vi "background writer.vi"(0 "dictionary":T1, 1 "command queue":refnum<k33>, 2 "response from processor":refnum<k33>, 3 "output type order":T3[](array[typedef]), 4 "File Property Indeces":i32[](array[numeric]), 5 "logging path":path, 7 "backup directory":path, 9 "cache allocation":T2, 10 "LogRotate":refnum<class "LogRotate.lvclass">=refnum, 11 "scans per write":u16=20, 12 "dictionary group names":T1, 13 "enable channel (bool)":i32, 14 "has enable channel":bool) -> (15 "error out":errorcluster)   [LabVIEW 2015, in "TDMS datalogger runtime.lvclass"]
uses:
  TDMS datalogger runtime.lvclass
  <vilib>/NI/Tag Bus/tag/Data Type.ctl
  data cache.ctl
  <vilib>/NI/Tag Bus/dictionary/full data dictionary.ctl
  message to background process.ctl
  control enum.ctl
  <vilib>/NI/Tag Bus/table/data table.ctl
  response from background process.ctl
  response enum.ctl
  <vilib>/NI/LogRotate/LogRotate.lvclass
  writer state enum.ctl
  <vilib>/NI/Tag Bus/table/data table.lvlib
  <vilib>/NI/Tag Bus/tag/tag descriptor.lvclass
  <vilib>/NI/Tag Bus/dictionary/data dictionary.lvclass
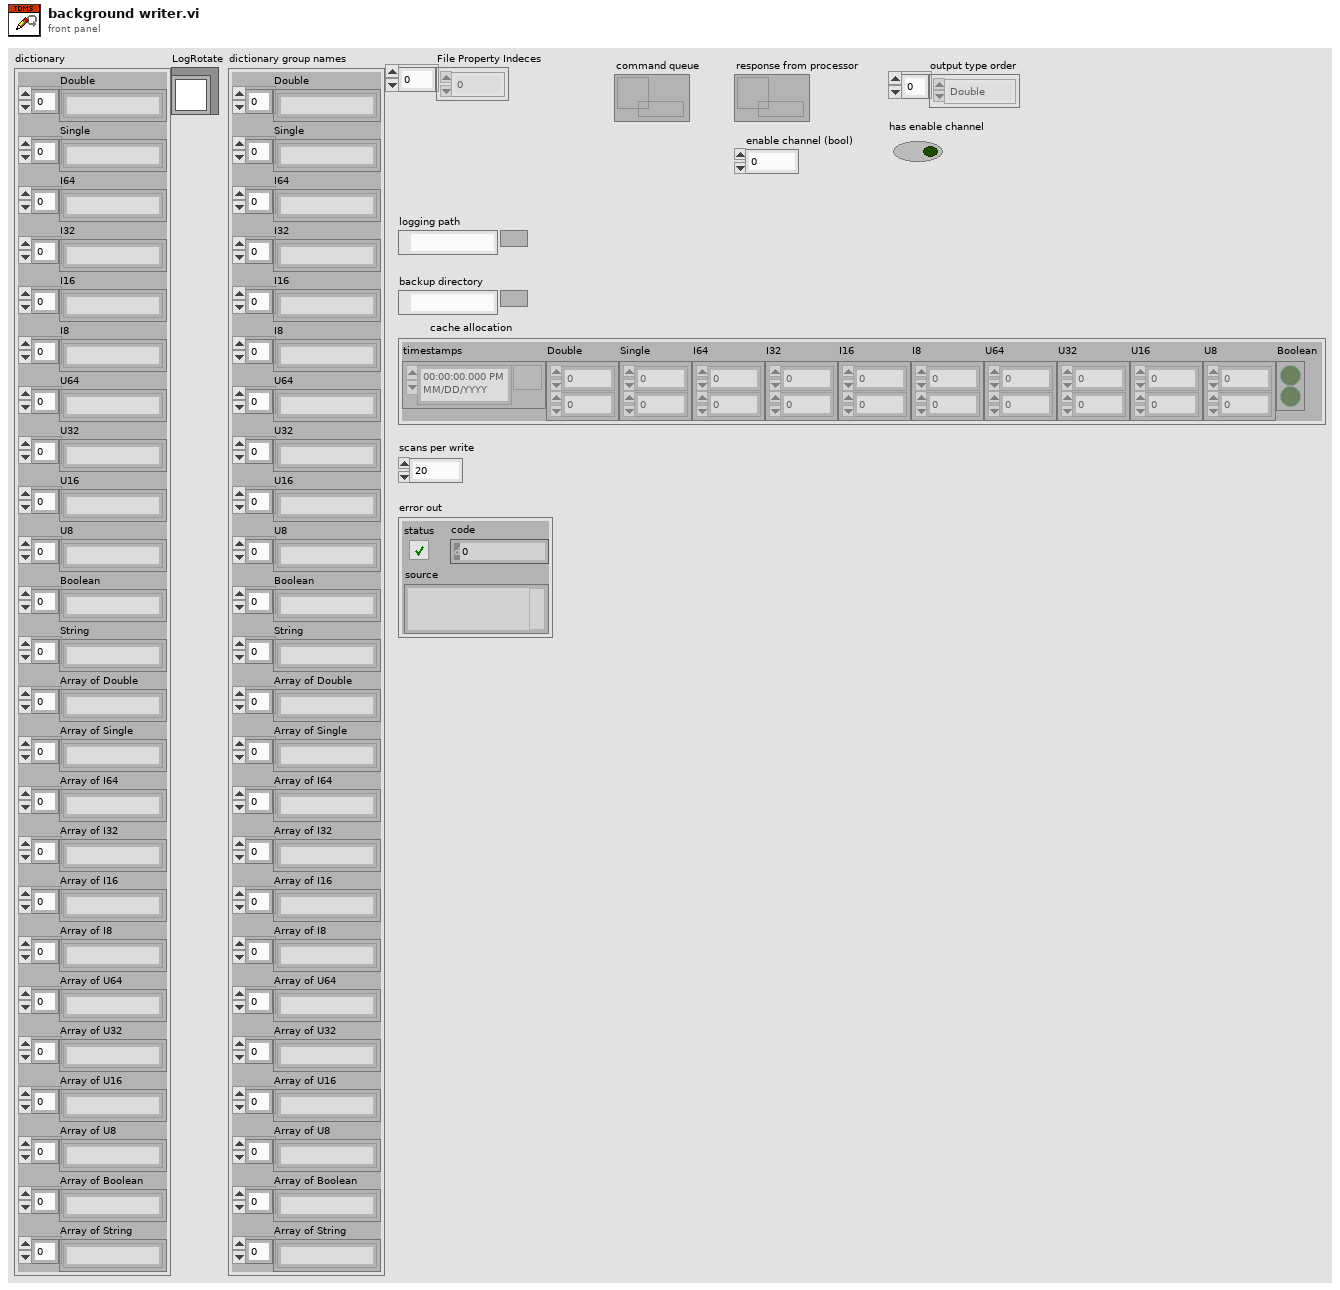
[diagram p1: front panel]
types:
  T1 = typedef "tag bus.lvlib/data dictionary.lvclass/full data dictionary.ctl" = cluster{"Double":string[], "Single":string[], "I64":string[], "I32":string[], "I16":string[], "I8":string[], "U64":string[], "U32":string[], "U16":string[], "U8":string[], "Boolean":string[], "String":string[], "Array of Double":string[], "Array of Single":string[], "Array of I64":string[], "Array of I32":string[], "Array of I16":string[], "Array of I8":string[], "Array of U64":string[], "Array of U32":string[], "Array of U16":string[], "Array of U8":string[], "Array of Boolean":string[], "Array of String":string[]}
  T2 = typedef "TDMS datalogger runtime.lvclass/data cache.ctl" = cluster{"timestamps":timestamp[], "Double":dbl[][], "Single":sgl[][], "I64":i64[][], "I32":i32[][], "I16":i16[][], "I8":i8[][], "U64":u64[][], "U32":u32[][], "U16":u16[][], "U8":u8[][], "Boolean":bool[][]}
  T3 = typedef "tag bus.lvlib/tag descriptor.lvclass/Data Type.ctl" = enum16{"Double", "Single", "I64", "I32", "I16", "I8", "U64", "U32", "U16", "U8", "Boolean", "String", "Array of Double", "Array of Single", "Array of I64", "Array of I32", "Array of I16", "Array of I8", "Array of U64", "Array of U32", "Array of U16", "Array of U8", "Array of Boolean", "Array of String"}
  T4 = typedef "TDMS datalogger runtime.lvclass/writer state enum.ctl" = enum16{"wait for message", "report error", "exit", "close file"}
  T5 = typedef "TDMS datalogger runtime.lvclass/response enum.ctl" = enum16{"exit", "return buffer", "error"}
  T6 = typedef "TDMS datalogger runtime.lvclass/response from background process.ctl" = cluster{"response enum":T5, "datapack":refnum<data-value>, "error code":i32}
  T7 = typedef "TDMS datalogger runtime.lvclass/message to background process.ctl" = cluster{"control enum":T8, "datapack":refnum<data-value>, "Time Stamp":timestamp}
  T8 = typedef "TDMS datalogger runtime.lvclass/control enum.ctl" = enum16{"exit", "output data"}
  T9 = typedef "tag bus.lvlib/data table.lvlib/data table.ctl" = cluster{"Double":dbl[], "Single":sgl[], "I64":i64[], "I32":i32[], "I16":i16[], "I8":i8[], "U64":u64[], "U32":u32[], "U16":u16[], "U8":u8[], "Boolean":bool[], "String":string[], "Array of Double":cluster{"DBL Array":dbl[]}[], "Array of Single":cluster{"SGL Array":sgl[]}[], "Array of I64":cluster{"I64 Array":i64[]}[], "Array of I32":cluster{"I32 Array":i32[]}[], "Array of I16":cluster{"I16 Array":i16[]}[], "Array of I8":cluster{"I8 Array":i8[]}[], "Array of U64":cluster{"U64 Array":u64[]}[], "Array of U32":cluster{"U32 Array":u32[]}[], "Array of U16":cluster{"U16 Array":u16[]}[], "Array of U8":cluster{"U8 Array":u8[]}[], "Array of Boolean":cluster{"Boolean Array":bool[]}[], "Array of String":cluster{"String Array":string[]}[]}
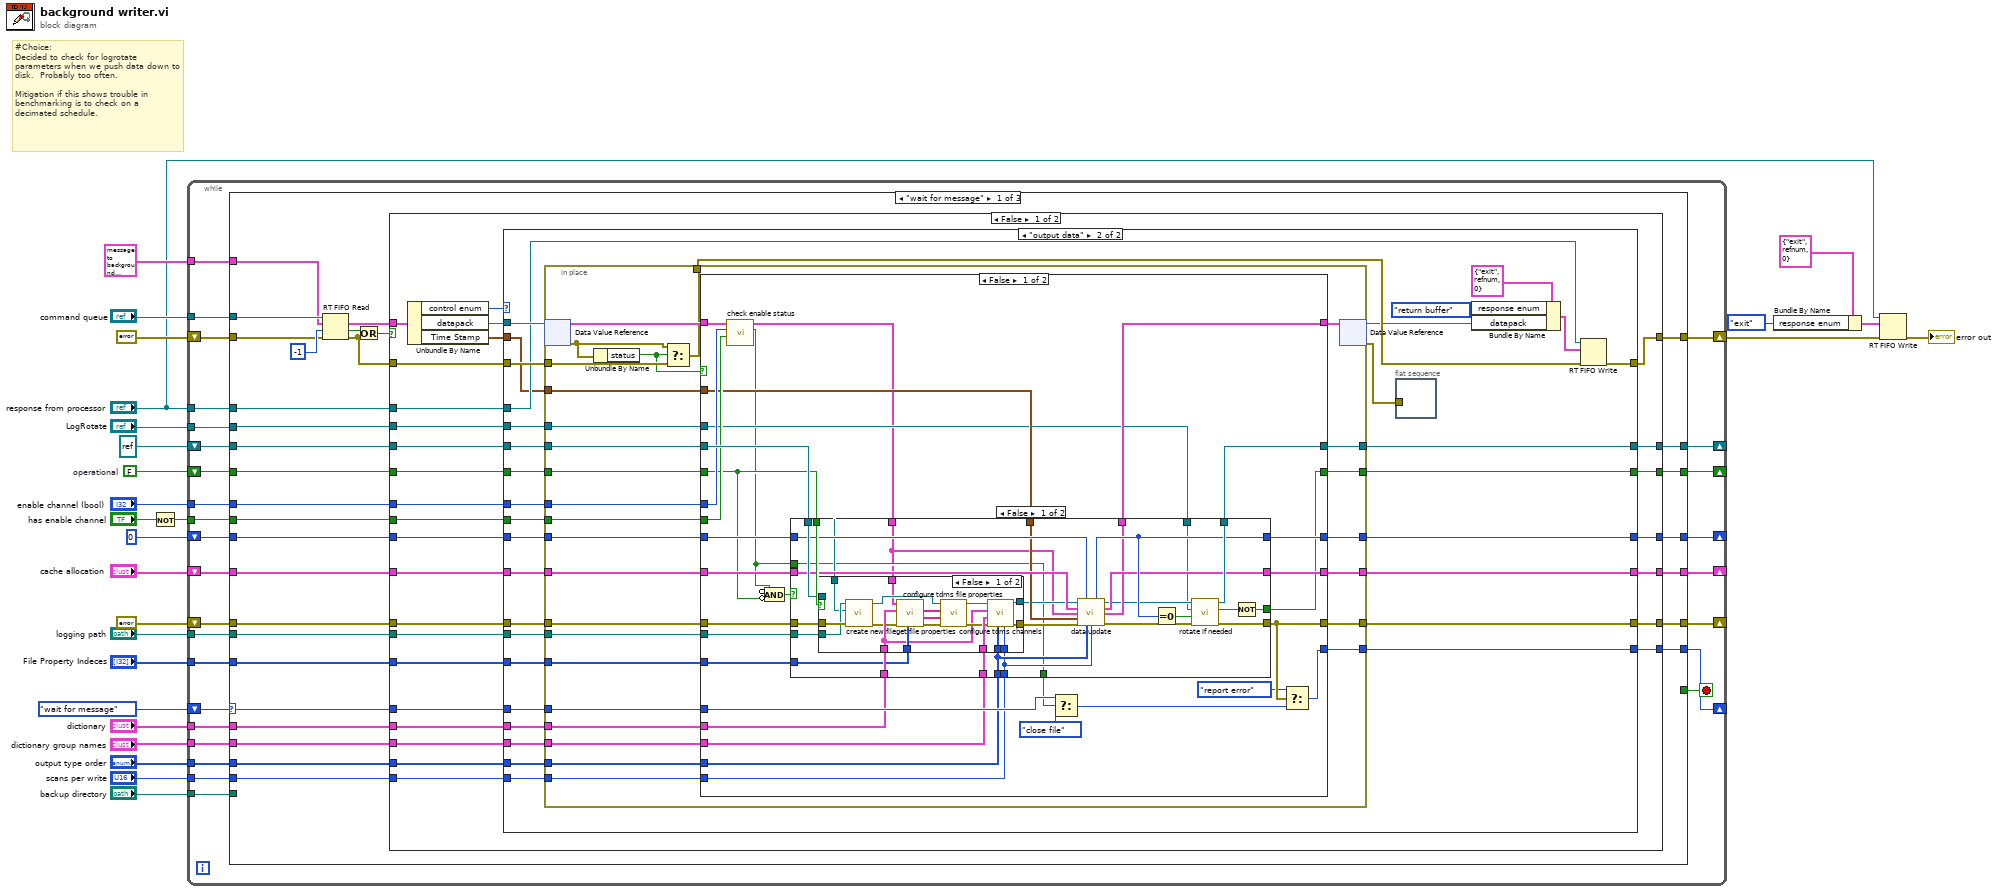
[diagram p0: block diagram]
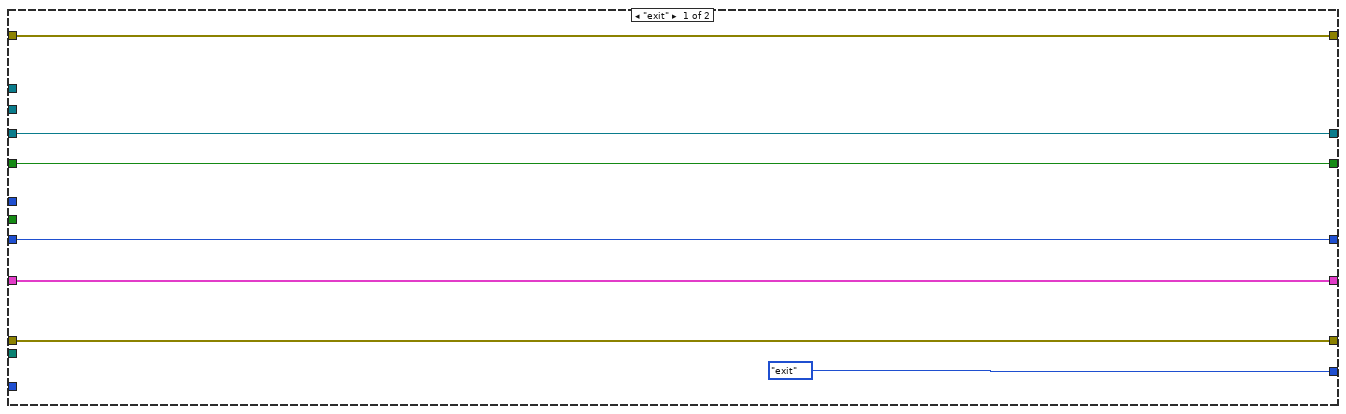
[diagram p2: hidden frame]
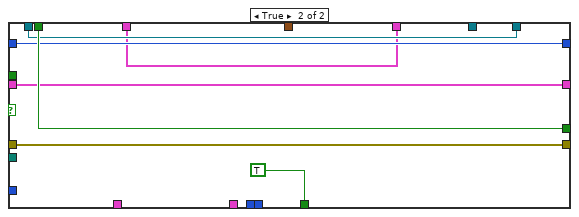
[diagram p4: hidden frame]
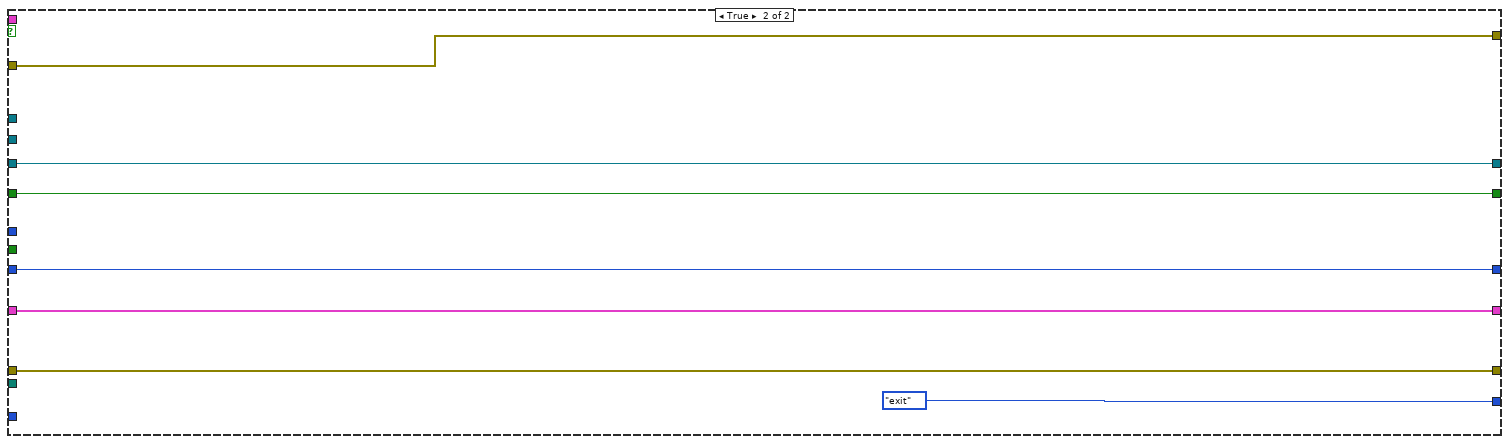
[diagram p6: hidden frame]
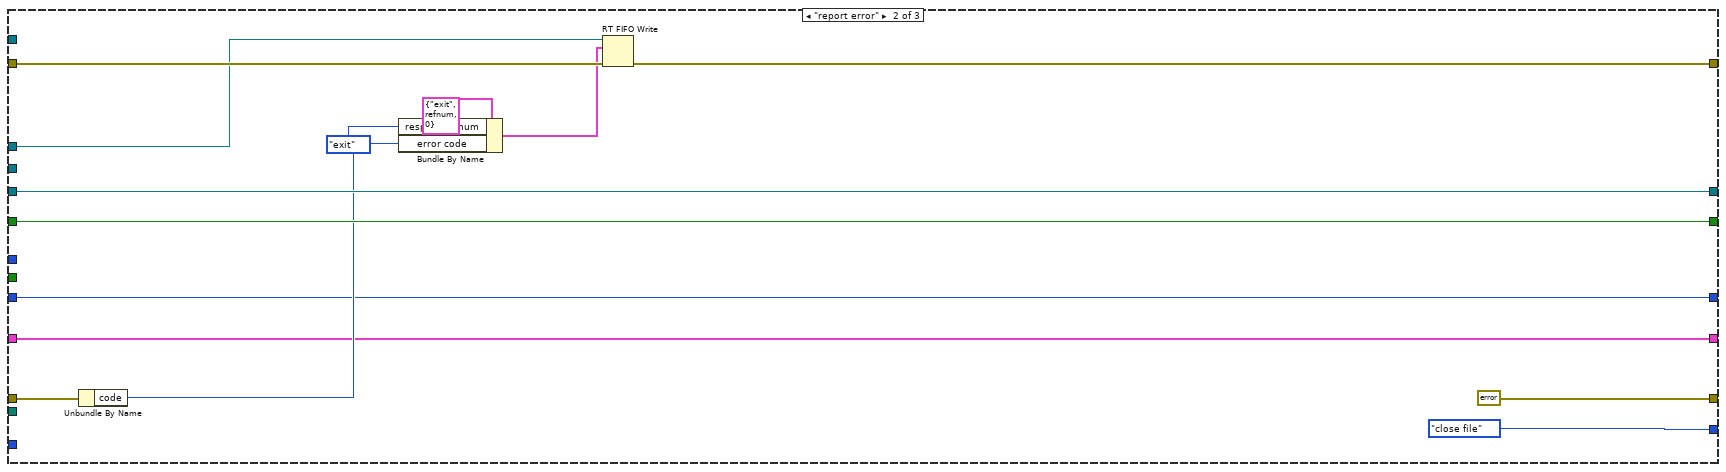
[diagram p7: hidden frame]
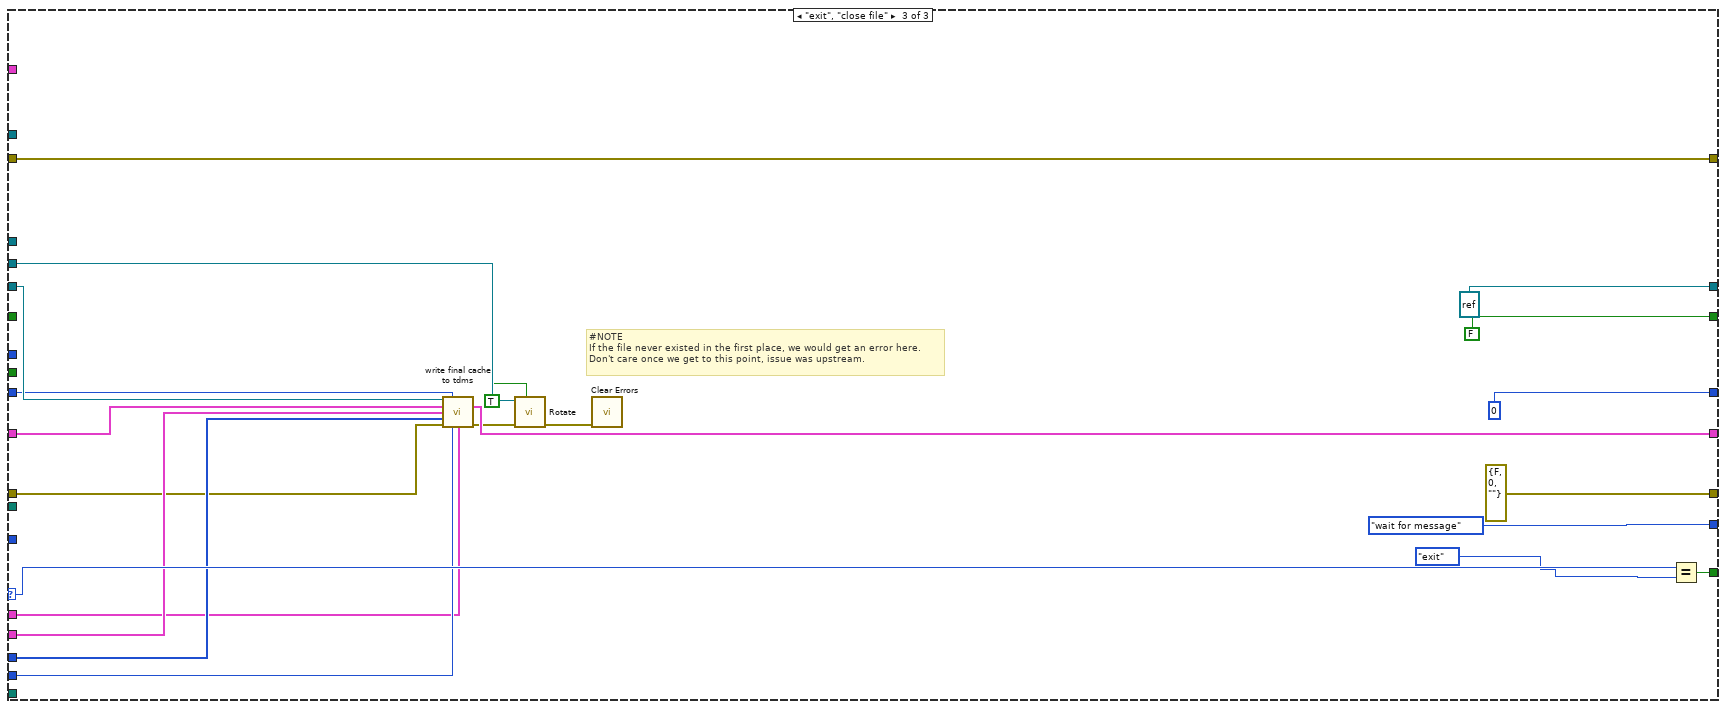
[diagram p8: hidden frame]
diagram:
  w15 = FALSE  # operational
  # "#Choice:\nDecided to check for logrotate parameters when we push data down to disk.  Probably too often.\n\nMitigation if this shows trouble in benchmarking is to check on a decimated schedule."
  n1 = Not(x="has enable channel") -> (.not. x?=w7:bool)
  n2 = while {
    tunnel: "command queue" -> [w54]
    tunnel: T7 {"control enum"=enum."exit", "datapack"=refnum, "Time Stamp"=timestamp(0 s since 1904-01-01)} ("element") -> [w53]
    shift-right: [w51] -> w23
    shift-left: errorcluster {"status"=FALSE, "code"=0, "source"=""} ("error in") -> [w52]
    tunnel: "response from processor" -> [w49]
    shift-right: [w47] -> _
    shift-left: writer_state_enum."wait for message" ("logger state") -> [w48]
    shift-right: [w45] -> _
    shift-left: refnum<k34> refnum ("tdms file out") -> [w46]
    shift-right: [w36] -> _
    shift-left: w15 -> [w44]
    shift-right: [w42] -> _
    shift-left: errorcluster {"status"=FALSE, "code"=0, "source"=""} ("error in") -> [w43]
    tunnel: "logging path" -> [w41]
    tunnel: "dictionary" -> [w40]
    tunnel: "output type order" -> [w39]
    tunnel: "scans per write" -> [w38]
    tunnel: "backup directory" -> [w37]
    shift-right: [w35] -> _
    shift-left: 0 ("sample counter") -> [w34]
    shift-right: [w29] -> _
    shift-left: "cache allocation" -> [w30]
    tunnel: "enable channel (bool)" -> [w32]
    tunnel: w7 -> [w33]
    tunnel: "dictionary group names" -> [w31]
    tunnel: "LogRotate" -> [w28]
    tunnel: "File Property Indeces" -> [w27]
    stop <- w50 stop-if-true
    n3 = case shown="\"wait for message\"" w48 {
      selector: w48 -> [w64 _ w313]
      tunnel: w54 -> [w85 _ _]
      tunnel: w53 -> [w83 _ _]
      tunnel: w52 -> [w82 w293 w315]
      tunnel: [w78 w291 w315] -> w51
      tunnel: [_ _ w314] -> w50
      tunnel: w49 -> [w76 w290 _]
      tunnel: [w75 writer_state_enum."close file" ("logger state") writer_state_enum."wait for message" ("logger state")] -> w47
      tunnel: w46 -> [w74 w292 w306]
      tunnel: [w73 w292 refnum<k34> refnum ("tdms file out")] -> w45
      tunnel: w44 -> [w71 w284 _]
      tunnel: w43 -> [w69 w283 w298]
      tunnel: [w70 errorcluster {"status"=FALSE, "code"=0, "source"=""} ("error out") errorcluster {"status"=FALSE, "code"=0, "source"=""} ("error out")] -> w42
      tunnel: w41 -> [w58 _ _]
      tunnel: w40 -> [w56 _ w300]
      tunnel: w39 -> [w61 _ w303]
      tunnel: w38 -> [w60 _ w301]
      tunnel: w37 -> [_ _ _]
      tunnel: [w72 w284 FALSE] -> w36
      tunnel: [w67 w280 0 ("sample counter")] -> w35
      tunnel: w34 -> [w68 w280 w302]
      tunnel: w33 -> [w62 _ _]
      tunnel: w32 -> [w63 _ _]
      tunnel: w31 -> [w57 _ w304]
      tunnel: w30 -> [w66 w281 w305]
      tunnel: [w65 w281 w299] -> w29
      tunnel: w28 -> [w59 _ w295]
      tunnel: w27 -> [w55 _ _]
      frame "wait for message" {
        n4 = RT FIFO Read(0:w85, 1:w83, 2:-1 ("timeout in ms (0)"), 3:w82) -> (9:w77:T7, 10:w81:bool, 11:w79:errorcluster)  [unwired: 2 out]
        n5 = Or(x=w81, y=w79) -> (x .or. y?=w80:bool)
        n6 = case shown="False" w80 {
          tunnel: w79 -> [w110 w279]
          tunnel: [w111 w279] -> w78
          tunnel: w77 -> [w113 _]
          tunnel: w76 -> [w107 _]
          tunnel: [w106 writer_state_enum."exit" ("logger state")] -> w75
          tunnel: w74 -> [w105 w277]
          tunnel: [w104 w277] -> w73
          tunnel: [w102 w276] -> w72
          tunnel: w71 -> [w103 w276]
          tunnel: [w101 w275] -> w70
          tunnel: w69 -> [w100 w275]
          tunnel: w68 -> [w98 w274]
          tunnel: [w99 w274] -> w67
          tunnel: w66 -> [w97 w273]
          tunnel: [w96 w273] -> w65
          tunnel: w64 -> [w95 _]
          tunnel: w63 -> [w94 _]
          tunnel: w62 -> [w93 _]
          tunnel: w61 -> [w92 _]
          tunnel: w60 -> [w91 _]
          tunnel: w59 -> [w90 _]
          tunnel: w58 -> [w89 _]
          tunnel: w57 -> [w88 _]
          tunnel: w56 -> [w87 _]
          tunnel: w55 -> [w86 _]
          frame False {
            n7 = Unbundle By Name(w113) -> ("control enum"=w112:T8, "datapack"=w108:refnum<data-value>, "Time Stamp"=w109:timestamp)
            n8 = case shown="\"output data\"" w112 {
              tunnel: [w120 w136] -> w111
              tunnel: w110 -> [w120 w151]
              tunnel: w109 -> [_ w128]
              tunnel: w108 -> [_ w152]
              tunnel: w107 -> [_ w133]
              tunnel: [writer_state_enum."exit" ("logger state") w140] -> w106
              tunnel: w105 -> [w118 w150]
              tunnel: [w118 w149] -> w104
              tunnel: w103 -> [w117 w147]
              tunnel: [w117 w148] -> w102
              tunnel: [w116 w141] -> w101
              tunnel: w100 -> [w116 w142]
              tunnel: [w114 w145] -> w99
              tunnel: w98 -> [w114 w146]
              tunnel: w97 -> [w115 w143]
              tunnel: [w115 w144] -> w96
              tunnel: w95 -> [_ w139]
              tunnel: w94 -> [_ w138]
              tunnel: w93 -> [_ w137]
              tunnel: w92 -> [_ w127]
              tunnel: w91 -> [_ w126]
              tunnel: w90 -> [_ w125]
              tunnel: w89 -> [_ w124]
              tunnel: w88 -> [_ w123]
              tunnel: w87 -> [_ w122]
              tunnel: w86 -> [_ w121]
              frame "exit" {
              }
              frame "output data" {
                n9 = in-place {
                  in-place-border: w151 -> [w180]
                  in-place-border: w150 -> [w175]
                  in-place-border: [w174] -> w149
                  in-place-border: [w173] -> w148
                  in-place-border: w147 -> [w172]
                  in-place-border: w146 -> [w171]
                  in-place-border: [w170] -> w145
                  in-place-border: [w169] -> w144
                  in-place-border: w143 -> [w168]
                  in-place-border: w142 -> [w167]
                  in-place-border: [w166] -> w141
                  in-place-border: [w165] -> w140
                  in-place-border: w139 -> [w164]
                  in-place-border: [w163] -> w135
                  in-place-border: w138 -> [w162]
                  in-place-border: w137 -> [w161]
                  in-place-border: w128 -> [w160]
                  in-place-border: w127 -> [w159]
                  in-place-border: w126 -> [w158]
                  in-place-border: w125 -> [w157]
                  in-place-border: w124 -> [w156]
                  in-place-border: w123 -> [w155]
                  in-place-border: w122 -> [w154]
                  in-place-border: w121 -> [w153]
                  n10 = in-place-dvr #1(w152) -> (w176:T9, w179:errorcluster)
                  n11 = Unbundle By Name(w179) -> ("status"=w178:bool)
                  n12 = Select(t=w179, s=w178, f=w180) -> (s? t:f=w163:errorcluster)
                  n13 = case shown="False" w178 {
                    tunnel: [w200 w272] -> w177
                    tunnel: w176 -> [w201 w272]
                    tunnel: w175 -> [w210 w271]
                    tunnel: [w211 w271] -> w174
                    tunnel: [w189 w270] -> w173
                    tunnel: w172 -> [w186 w270]
                    tunnel: w171 -> [w208 w269]
                    tunnel: [w209 w269] -> w170
                    tunnel: [w204 w268] -> w169
                    tunnel: w168 -> [w205 w268]
                    tunnel: w167 -> [w207 w267]
                    tunnel: [w206 w267] -> w166
                    tunnel: [w203 w266] -> w165
                    tunnel: w164 -> [w202 w266]
                    tunnel: w162 -> [w199 _]
                    tunnel: w161 -> [w198 _]
                    tunnel: w160 -> [w197 _]
                    tunnel: w159 -> [w196 _]
                    tunnel: w158 -> [w195 _]
                    tunnel: w157 -> [w188 _]
                    tunnel: w156 -> [w194 _]
                    tunnel: w155 -> [w193 _]
                    tunnel: w154 -> [w183 _]
                    tunnel: w153 -> [w182 _]
                    frame False {
                      n14 = call "check enable status.vi"("always enabled?"=w198, "enable channel index"=w199, "data table in"=w201) -> ("enabled?"=w185:bool, "Data table out"=w181:T9)  [unwired: 7 in]
                      n15 = Compound Arithmetic op=AND(invert w185, invert w186) -> (w187:bool)
                      n16 = case shown="False" w187 {
                        tunnel: w186 -> [w238 w264]
                        tunnel: [w237 w262] -> w211
                        tunnel: w210 -> [w236 w262]
                        tunnel: [w235 w263] -> w209
                        tunnel: w208 -> [w234 w263]
                        tunnel: w207 -> [w233 w265]
                        tunnel: [w232 w265] -> w206
                        tunnel: w205 -> [w231 w261]
                        tunnel: [w230 w261] -> w204
                        tunnel: [w229 w259] -> w200
                        tunnel: w197 -> [w228 _]
                        tunnel: w196 -> [w227 _]
                        tunnel: w195 -> [w226 _]
                        tunnel: w194 -> [w225 _]
                        tunnel: w193 -> [w224 _]
                        tunnel: w183 -> [w223 _]
                        tunnel: [w216 w264] -> w189
                        tunnel: w188 -> [w215 _]
                        tunnel: w185 -> [w214 _]
                        tunnel: [w214 TRUE ("enabled?")] -> w184
                        tunnel: w182 -> [w213 _]
                        tunnel: w181 -> [w212 w259]
                        frame False {
                          n17 = case shown="False" w238 {
                            tunnel: w236 -> [_ w257]
                            tunnel: w233 -> [w256 w258]
                            tunnel: [w255 w258] -> w219
                            tunnel: [w254 w257] -> w218
                            tunnel: w225 -> [w253 _]
                            tunnel: w224 -> [w249 _]
                            tunnel: w223 -> [w243 _]
                            tunnel: w227 -> [w252 _]
                            tunnel: w226 -> [w251 _]
                            tunnel: w215 -> [w250 _]
                            tunnel: w213 -> [w245 _]
                            tunnel: w212 -> [w244 _]
                            frame False {
                              n18 = call "create new file.vi"("error in"=w256, "LogRotate in"=w250, "logging path"=w253) -> ("error out"=w239:errorcluster, "tdms file out"=w248:refnum<k34>)  [unwired: 7 in]
                              n19 = call "get file properties.vi"("File Property Indeces"=w245, "error in"=w239, "dictionary"=w243, "data table in"=w244) -> ("error out"=w240:errorcluster, "File Property Values"=w241:string[], "File Property Names"=w242:string[])  [unwired: 4 in, 1 out]
                              n20 = call "configure tdms file properties.vi"("error in (no error)"=w240, "property values"=w241, "property names"=w242, "tdms file"=w248) -> ("error out"=w246:errorcluster, "tdms file out"=w247:refnum<k34>)  [unwired: 6 in]
                              n21 = call "configure tdms channels.vi"("samples per channel (1)"=w251, "type order"=w252, "error in"=w246, "dictionary group names"=w249, "dictionary"=w243, "tdms file in"=w247) -> ("error out"=w255:errorcluster, "tdms file out"=w254:refnum<k34>)  [unwired: 4 in]
                            }
                            frame True {
                            }
                          }
                          n22 = call "data update.vi"("tdms in"=w218, "sample counter in"=w234, "cache in"=w231, "data table in"=w212, "Time Stamp"=w228, "error in"=w219, "output type order"=w227, "scans per write"=w226) -> ("sample counter out"=w235:i32, "tdms out"=w221:refnum<k34>, "cache out"=w230:T2, "data table out"=w229:T9, "error out"=w222:errorcluster)  [unwired: 3 in]
                          n23 = Equal To 0?(x=w235) -> (x = 0?=w220:bool)
                          n24 = call "rotate if needed.vi"("error in"=w222, "Check?"=w220, "LogRotate"=w215, "tdms ref in"=w221) -> ("error out"=w232:errorcluster, "rotated?"=w217:bool, "tdms ref out"=w237:refnum<k34>)  [unwired: 5 in]
                          n25 = Not(x=w217) -> (.not. x?=w216:bool)
                        }
                        frame True {
                        }
                      }
                      n26 = Select(t=w202, s=w184, f=writer_state_enum."close file") -> (s? t:f=w190:T4)
                      n27 = Select(t=writer_state_enum."report error", s=w206, f=w190) -> (s? t:f=w203:T4)
                    }
                    frame True {
                    }
                  }
                  n28 = in-place-dvr #1(w177) -> (w130:refnum<data-value>, w134:errorcluster)
                }
                n29 = flat-sequence {
                  tunnel: w134 -> [_]
                  frame #0 {
                  }
                }
                n30 = Bundle By Name(cluster=T6 {"response enum"=enum."exit", "datapack"=refnum, "error code"=0} ("element"), "response enum"=response_enum."return buffer", "datapack"=w130) -> (w131:T6)
                n31 = RT FIFO Write(0:w133, 1:w131, 3:w135) -> (11:w136:errorcluster)  [unwired: 2 in, 3 out]
              }
            }
          }
          frame True {
          }
        }
      }
      frame "report error" {
        n32 = Unbundle By Name(w283) -> ("code"=w282:i32)
        n33 = Bundle By Name(cluster=T6 {"response enum"=enum."exit", "datapack"=refnum, "error code"=0} ("element"), "response enum"=response_enum."exit", "error code"=w282) -> (w288:T6)
        n34 = RT FIFO Write(0:w290, 1:w288, 3:w293) -> (11:w291:errorcluster)  [unwired: 2 in, 3 out]
      }
      frame "exit", "close file" {
        # "#NOTE\nIf the file never existed in the first place, we would get an error here.\nDon't care once we get to this point, issue was upstream."
        n35 = call "write final cache to tdms.vi"("tdms file in"=w306, "sample counter"=w302, "cache in"=w305, "dictionary group names"=w304, "output type order"=w303, "error in"=w298, "scans per write"=w301, "dictionary"=w300) -> ("cache out"=w299:T2, "error out"=w297:errorcluster)  [unwired: 6 in]
        n36 = call <vilib>:"Rotate.vi"("Force rotate"=TRUE, "error in (no error)"=w297, "LogRotate in"=w295) -> ("error out"=w296:errorcluster)  [unwired: 7 in, 1 out]
        n37 = call <vilib>:"Clear Errors.vi"("error in (no error)"=w296) -> ()  [unwired: 5 in, 2 out]
        n38 = Equal?(x=w313, y=writer_state_enum."exit") -> (x = y?=w314:bool)
      }
    }
  }
  n39 = Bundle By Name(cluster=T6 {"response enum"=enum."exit", "datapack"=refnum, "error code"=0} ("element"), "response enum"=response_enum."exit") -> (w20:T6)
  n40 = RT FIFO Write(0:"response from processor", 1:w20, 3:w23) -> (11:→"error out":errorcluster)  [unwired: 2 in, 3 out]
